vi "Single Tone Microphone Measurements (N Ch).vi"(6 "units settings":T2, 8 "error in":errorcluster, 10 "measurement settings":T4={"Band start"=20.0, "Band stop"=20000.0, "Frequency"=1000.0}, 11 "waveforms":waveform(dbl)[](array[waveform])) -> (0 "error out":errorcluster, 1 "spectra":cluster{"x0":dbl, "dx":dbl, "magnitude":dbl[]}[](array[cluster]), 2 "waveforms":waveform(dbl)[](array[waveform]), 3 "measurements":T1[](array[typedef]))   [LabVIEW 2022 SP3]
uses:
  controls/single tone microphone measurement settings.ctl
  controls/units settings - mic.ctl
  controls/measurement units.ctl
  controls/single tone microphone measurements.ctl
  <vilib>/addons/_NISVFA/_Shared subVIs/Common/SVL Set dB Reference (N Ch - 1 Ref).vi
  <vilib>/addons/_NISVFA/_Spectrum Processing/SVFA Unit Conversion (Complex) (1 Ch).vi
  <vilib>/addons/_NISVFA/_Shared subVIs/Common/SVL Set dB Reference (1 Ch).vi
  <vilib>/addons/_NISVFA/_Shared subVIs/Common/svc_Log View for Spectrum (1Ch).vi
  <vilib>/addons/_NISVFA/_Spectrum Processing/SVFA Unit Conversion (1 Ch).vi
  <vilib>/addons/_NISVFA/_Shared subVIs/Common/svc_Complex Datatype Defaults.vi
  <vilib>/addons/_NISVFA/_Shared subVIs/Common/SVL Set dB Reference (variant).vi
  <vilib>/addons/_NISVFA/_Shared subVIs/Common/svc_Unwrap Phase.vi
  <vilib>/addons/_NISVFA/_Shared subVIs/Common/svc_Convert Spectrum Array to dB.vi
  <vilib>/addons/_NISVFA/_Shared subVIs/Common/svc_Spectrum Units.vi
  <vilib>/addons/_NISVFA/_Spectrum Processing/subVIs/svfa_Conversion Utility (spectrum info).vi
  <vilib>/addons/_NISVFA/_Shared subVIs/Common/svc_Format Value (DBL).vi
  <vilib>/addons/_NISVFA/_Shared subVIs/Common/svc_Get Weighting Enum and Labels.vi
  <vilib>/addons/_NISVFA/_Shared subVIs/Common/svc_Engineering Units to Unit Label.vi
  <vilib>/addons/_NISVFA/_Shared subVIs/Common/svc_Surround NonAlpha String with Parentheses.vi
  <vilib>/dlg_ctls.llb/Space Constant.vi
  <vilib>/addons/_NISVFA/_Spectrum Processing/subVIs/svfa_Peak to RMS to Peak2Peak.vi
  <vilib>/addons/_NISVFA/_Spectrum Processing/subVIs/svfa_Mag to Mag2.vi
  <vilib>/addons/_NISVFA/_Spectrum Processing/subVIs/svfa_Linear to dB.vi
  <vilib>/addons/_NISVFA/_Spectrum Processing/subVIs/svfa_dBrefA to dBrefB.vi
  <vilib>/addons/_NISVFA/_Spectrum Processing/subVIs/svfa_Spectrum to Spectral Density.vi
  <vilib>/addons/_NISVFA/_Shared subVIs/Common/svc_Unit Label Lexical Class.vi
  <vilib>/addons/_NISVFA/_Shared subVIs/Common/svc_Window Parameters.vi
  <vilib>/addons/_NISVFA/_Shared subVIs/Common/svc_Caller VI Returned in Error Source.vi
  <vilib>/addons/Sound and Vibration/svt_Level/SVL Leq Sound Level (1 Ch).vi
  <vilib>/addons/Sound and Vibration/svt_Distortion/SVT SNR without Harmonics (Time) (1 Ch).vi
  <vilib>/addons/_NISVFA/_Spectrum Processing/SVFA Extract Single Tone Information (Complex) (1 Ch).vi
  <vilib>/Analysis/4window.llb/window parameters.vi
  <vilib>/Analysis/4window.llb/Window Properties.vi
  <vilib>/Analysis/4window.llb/Window Properties by Name.vi
  <vilib>/addons/Sound and Vibration/svt_Distortion/SoundVib_Distortion.lvlib
  <vilib>/addons/Sound and Vibration/svt_Level/SoundVib_SoundLevel.lvlib
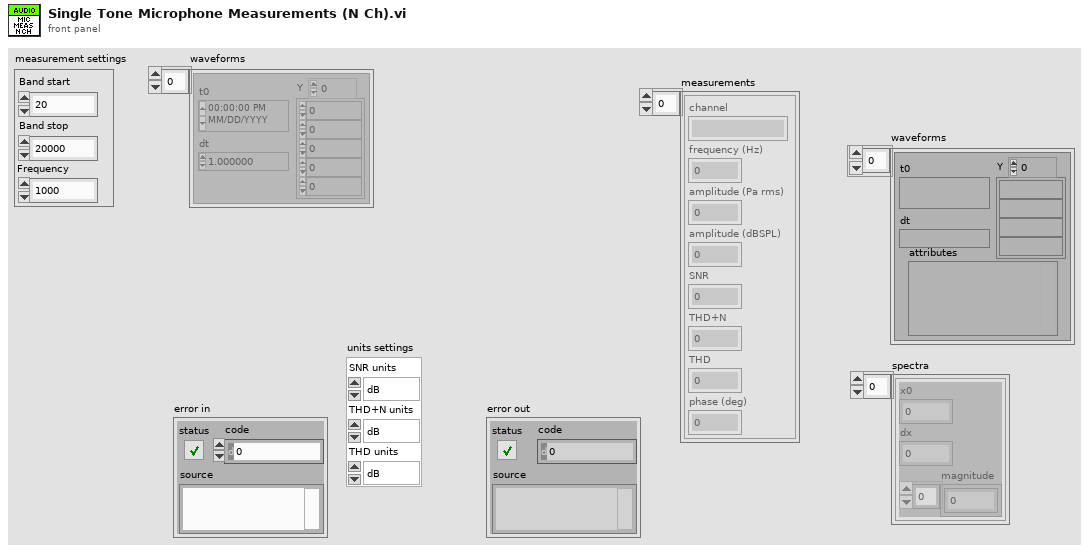
[diagram p1: front panel]
types:
  T1 = typedef "single tone microphone measurements.ctl" = cluster{"channel":string, "frequency (Hz)":dbl, "amplitude (Pa rms)":dbl, "amplitude (dBSPL)":dbl, "SNR":dbl, "THD+N":dbl, "THD":dbl, "phase (deg)":dbl}
  T2 = typedef "units settings - mic.ctl" = cluster{"SNR units":T3, "THD+N units":T3, "THD units":T3}
  T3 = typedef "measurement units.ctl" = enum32{"dB", "%", "x/y"}
  T4 = typedef "single tone microphone measurement settings.ctl" = cluster{"Band start":dbl, "Band stop":dbl, "Frequency":dbl}
  T5 = cluster{"start frequency":dbl, "stop frequency":dbl}
  T6 = cluster{"SNR units":enum16{"dB", "linear ratio", "%"}, "detected fundamental amplitude units":enum16{"EU rms", "EU peak", "EU peak-peak"}}
  T7 = enum16{"no change", "spectrum", "spectral density"}
  T8 = cluster{"linear/dB":enum16{"no change", "linear", "dB"}, "dB reference (0: no change)":dbl, "power/magnitude":enum16{"no change", "power", "magnitude"}, "view":enum16{"no change", "rms", "peak", "peak-peak"}}
  T9 = typedef "svc_Spectrum Info.ctl" = cluster{"channel name":string, "description":string, "x-axis units":T10, "spectral info":cluster{"spectrum type":T11, "linear/dB":enum16{"linear", "dB"}, "window":u16, "window size":i32, "FFT size":i32}, "engineering units":T12, "custom label":string, "dB reference [EU]":dbl, "peak units":enum16{"rms", "peak", "peak-peak"}, "weighting filter":T13, "spectral density?":bool, "unit label":string, "spectrum skewed?":bool, "complimentary spectrum units":T14}
  T10 = typedef "svc_X-Axis Units.ctl" = u16
  T11 = typedef "svc_Spectrum Type.ctl" = enum16{"FFT Spectrum [complex]", "Amplitude [Magnitude]", "Power [Magnitude^2]", "Cross Spectrum [complex]", "Frequency Response [Complex]"}
  T12 = typedef "svc_Engineering Units Text Ring.ctl" = u16
  T13 = typedef "svc_Weighting Filter Text Ring.ctl" = u16
  T14 = typedef "svc_Complimentary Spectrum Units.ctl" = enum16{"none", "radians", "degrees", "cycles", "imaginary"}
  T15 = cluster{"complex spectrum response":cluster{"f0":dbl, "df":dbl, "complex spectrum":cdb[]}, "spectrum info":T9}
  T16 = cluster{"frequency [Hz]":dbl, "amplitude [EU pk]":dbl, "phase (deg)":dbl}
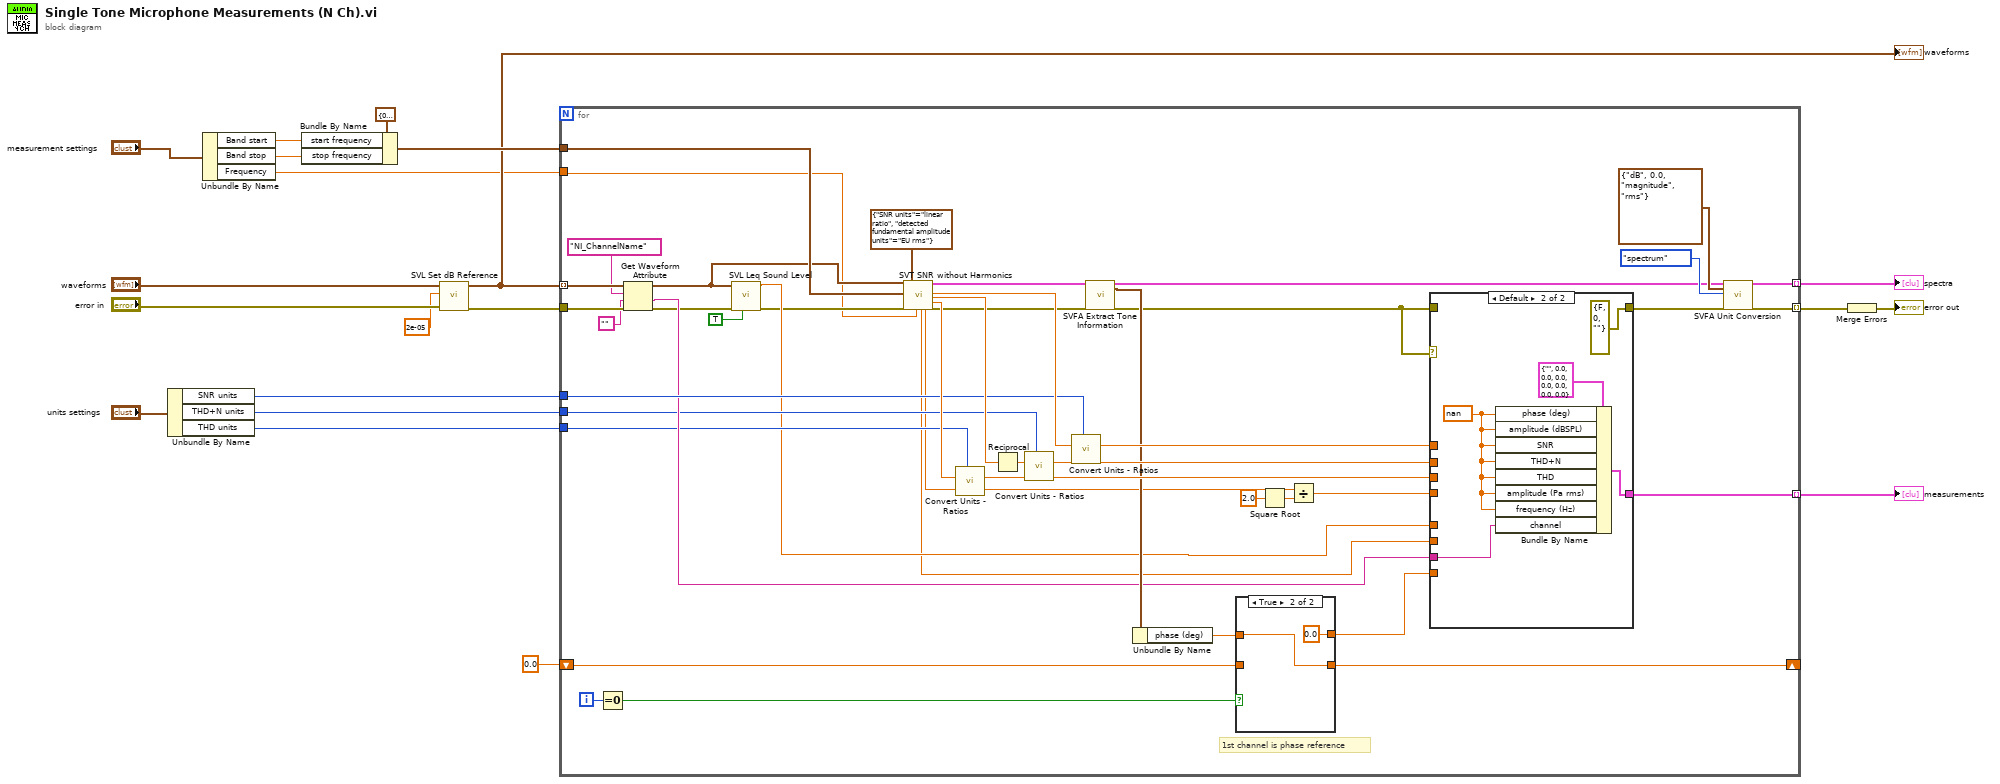
[diagram p0: block diagram]
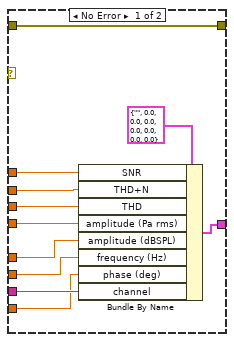
[diagram p2: hidden frame]
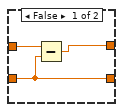
[diagram p3: hidden frame]
diagram:
  n1 = Unbundle By Name("units settings") -> ("SNR units"=w4:T3, "THD+N units"=w12:T3, "THD units"=w11:T3)
  n2 = Unbundle By Name("measurement settings") -> ("Band start"=w19:dbl, "Band stop"=w20:dbl, "Frequency"=w1:dbl)
  n3 = Bundle By Name(cluster=T5 {"start frequency"=0.0, "stop frequency"=0.0} ("frequency range"), "start frequency"=w19, "stop frequency"=w20) -> (w17:T5)
  n4 = call-poly <vilib>:"SVL Set dB Reference.vi"("error in (no error)"="error in", "dB reference [EU]"=2e-05, "scaled signals in [EU]"="waveforms") -> ("error out"=w15:errorcluster, "scaled signals out [EU]"=w9:waveform(dbl)[])  [unwired: 7 in]
  "waveforms" <- w9
  n5 = for {
    tunnel: w17 -> [w62]
    tunnel: [w61] -> w2 mode=indexing
    tunnel: w12 -> [w32]
    tunnel: w11 -> [w33]
    tunnel: w4 -> [w53]
    tunnel: [w34] -> w7 mode=indexing
    tunnel: w9 -> [w41] mode=indexing
    shift-right: [w43] -> _
    shift-left: 0.0 -> [w45]
    tunnel: w15 -> [w40]
    tunnel: [w35] -> w5 mode=indexing
    tunnel: w1 -> [w21]
    i -> [w47]
    # "1st channel is phase reference"
    n6 = Equal To 0?(x=w47) -> (x = 0?=w46:bool)
    n7 = Get Waveform Attribute(4:w40, 5:"", 6:"NI_ChannelName" ("name"), 7:w41) -> (0:w30:errorcluster, 1:w37:string, 3:w22:waveform(dbl))  [unwired: 1 out]
    n8 = call-poly <vilib>:"SVL Leq Sound Level.vi"("restart averaging (F)"=TRUE, "error in (no error)"=w30, "scaled signal [EU]"=w22) -> ("error out"=w23:errorcluster, "Leq sound level [dB EU]"=w28:dbl)  [unwired: 6 in, 1 out]
    n9 = call-poly <vilib>:"SVT SNR without Harmonics.vi"("scaled signal [EU]"=w22, "frequency range"=w62, "error in (no error)"=w23, "desired units"=T6 {"SNR units"=enum."linear ratio", "detected fundamental amplitude units"=enum."EU rms"}, "expected fundamental frequency [Hz]"=w21) -> ("detected fundamental\nfrequency [Hz]"=w25:dbl, "detected fundamental\namplitude"=w24:dbl, "complex spectrum"=w31:T15, "SNR (without harmonics)"=w60:dbl, "SINAD"=w57:dbl, "THD"=w55:dbl, "error out"=w49:errorcluster)  [unwired: 7 in, 1 out]
    n10 = call "Convert Units - Ratios.vi"("units"=w33, "linear ratio"=w55) -> ("converted ratio"=w54:dbl)  [unwired: 9 in]
    n11 = Reciprocal(x=w57) -> (1/x=w58:dbl)
    n12 = call "Convert Units - Ratios.vi"("units"=w32, "linear ratio"=w58) -> ("converted ratio"=w56:dbl)  [unwired: 9 in]
    n13 = call "Convert Units - Ratios.vi"("units"=w53, "linear ratio"=w60) -> ("converted ratio"=w59:dbl)  [unwired: 9 in]
    n14 = call-poly <vilib>:"SVFA Extract Tone Information.vi"("complex spectrum"=w31, "error in"=w49) -> ("complex spectrum"=w27:T15, "detected tone"=w48:T16, "error out"=w26:errorcluster)  [unwired: 14 in, 1 out]
    n15 = Unbundle By Name(w48) -> ("phase (deg)"=w44:dbl)
    n16 = case shown="True" w46 {
      tunnel: w45 -> [w83 _]
      tunnel: w44 -> [w84 w86]
      tunnel: [w82 0.0] -> w42
      tunnel: [w83 w86] -> w43
      frame False {
        n17 = Subtract(x=w84, y=w83) -> (x-y=w82:dbl)
      }
      frame True {
      }
    }
    n18 = Square Root(x=2.0 ("y")) -> (sqrt(x)=w52:dbl)
    n19 = Divide(x=w24, y=w52) -> (x/y=w50:dbl)
    n20 = case shown="Default" w26 {
      tunnel: [w75 w80] -> w61
      tunnel: w59 -> [w74 _]
      tunnel: w56 -> [w73 _]
      tunnel: w54 -> [w72 _]
      tunnel: w25 -> [w69 _]
      tunnel: w50 -> [w71 _]
      tunnel: w42 -> [w67 _]
      tunnel: w37 -> [w68 w79]
      tunnel: w26 -> [w70 _]
      tunnel: [w70 errorcluster {"status"=FALSE, "code"=0, "source"=""} ("error out")] -> w36
      tunnel: w28 -> [w66 _]
      frame No Error {
        n21 = Bundle By Name(cluster=T1 {"channel"="", "frequency (Hz)"=0.0, "amplitude (Pa rms)"=0.0, "amplitude (dBSPL)"=0.0, "SNR"=0.0, "THD+N"=0.0, "THD"=0.0, "phase (deg)"=0.0} ("results"), "SNR"=w74, "THD+N"=w73, "THD"=w72, "amplitude (Pa rms)"=w71, "amplitude (dBSPL)"=w66, "frequency (Hz)"=w69, "phase (deg)"=w67, "channel"=w68) -> (w75:T1)
      }
      frame Default {
        w77 = nan ("SFDR (dBc)")
        n22 = Bundle By Name(cluster=T1 {"channel"="", "frequency (Hz)"=0.0, "amplitude (Pa rms)"=0.0, "amplitude (dBSPL)"=0.0, "SNR"=0.0, "THD+N"=0.0, "THD"=0.0, "phase (deg)"=0.0} ("results"), "phase (deg)"=w77, "amplitude (dBSPL)"=w77, "SNR"=w77, "THD+N"=w77, "THD"=w77, "amplitude (Pa rms)"=w77, "frequency (Hz)"=w77, "channel"=w79) -> (w80:T1)
      }
    }
    n23 = call-poly <vilib>:"SVFA Unit Conversion.vi"("complex spectrum"=w27, "desired scaling"=T8 {"linear/dB"=enum."dB", "dB reference (0: no change)"=0.0, "power/magnitude"=enum."magnitude", "view"=enum."rms"}, "spectral density desired"=T7."spectrum", "error in (no error)"=w36) -> ("converted spectrum"=w34:cluster{"x0":dbl, "dx":dbl, "magnitude":dbl[]}, "error out"=w35:errorcluster)  [unwired: 10 in, 4 out]
  }
  "spectra" <- w7
  "measurements" <- w2
  n24 = Merge Errors(w5) -> (→"error out":errorcluster)
